vi "Fit To Pane.vi"() -> ()   [LabVIEW 2020]
doc: "Development tool: makes a control fill its pane of a splitter panel and keep filling it (what Fit Control to Pane does by hand). The pane is scrolled to 0,0 and the control moved there; with scaling off, the pane is shrunk to the control's size by moving the two splitter bars that bound it (the window is not resized: writing Panel Bounds answered error 1 once a second pane scaled an object); Scale Single Object is switched on for the control and the bars are put back, so the control grows with the pane and fills it exactly. Works for controls without a writable size (subpanels, multicolumn listboxes). Cell Width > 0 first sizes a multicolumn listbox: the first column's width, one visible column, the number of visible rows, no column headers and no vertical scroll bar; the bars then only make up the last pixels (a bar that would make a pane smaller than its minimum answers error 1358). Height Bar -1: no bar sets the pane's height (a pane beside a vertical bar that runs the full height of the window). Run it on a VI that is not running; it saves the VI (closing the last reference would unload it and drop the changes)."
panel:
  out "error out":errorcluster
  out "pane size":i32[](array[numeric])
  out "control size":i32[](array[numeric])
  in  "Rows":i32
  in  "Row Height":i32
  in  "Cell Width":i32
  in  "Height Bar":i32=1
  in  "Pane Left Of Bar":bool
  in  "Width Bar":i32
  in  "Label":string
  in  "VI":path
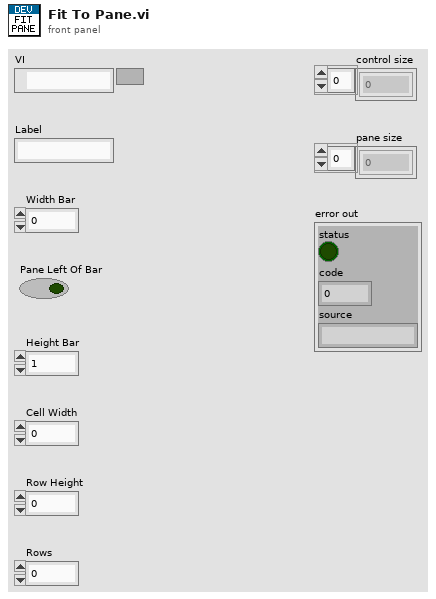
[diagram p1: front panel]
types:
  T1 = enum16{"No Scaling", "Scale All Objects", "Scale Single Object"}
  T2 = typedef "LVBoundsTypeDef.ctl" = cluster{"Width":u32, "Height":u32}
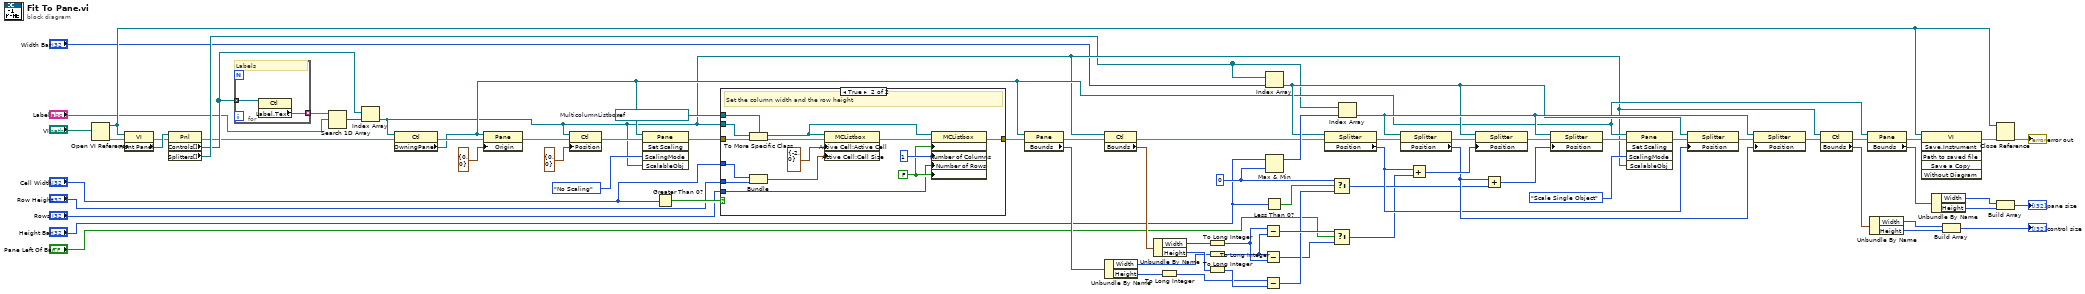
[diagram p0: block diagram]
diagram:
  w63 = refnum<vi> refnum  # MulticolumnListbox
  w46 = 0
  n1 = Open VI Reference(vi path="VI") -> (vi reference=w9:refnum<vi>, error out=w10:errorcluster)  [unwired: 5 in]
  n2 = property class="VI"(reference=w9, error in=w10) -> (error out=w11:errorcluster, "Front Panel"=w12:refnum<vi>)  [unwired: 1 out]
  n3 = property class="Pnl"(reference=w12, error in=w11) -> (error out=w13:errorcluster, "Controls[]"=w14:refnum<vi>[], "Splitters[]"=w15:refnum<vi>[])  [unwired: 1 out]
  n4 = for {
    tunnel: w14 -> [w76] mode=indexing
    tunnel: [w77] -> w16 mode=indexing
    # "Labels"
    n5 = property class="Ctl"(reference=w76) -> ("Label.Text"=w77:string)  [unwired: 1 in, 2 out]
  }
  n6 = Search 1D Array(1D array=w16, element="Label") -> (index of element=w17:i32)  [unwired: 1 in]
  n7 = Index Array(array=w14, index=w17) -> (element=w18:refnum<vi>)
  n8 = property class="Ctl"(reference=w18, error in=w13) -> (error out=w20:errorcluster, "OwningPane"=w19:refnum<vi>)  [unwired: 1 out]
  n9 = property class="Pane"(reference=w19, error in=w20, "Origin"=cluster{"Horizontal":i16, "Vertical":i16} {"Horizontal"=0, "Vertical"=0}) -> (error out=w22:errorcluster)  [unwired: 1 out]
  n10 = property class="Ctl"(reference=w18, error in=w22, "Position"=cluster{"Left":i32, "Top":i32} {"Left"=0, "Top"=0}) -> (error out=w24:errorcluster)  [unwired: 1 out]
  n11 = invoke class="Pane" method="Set Scaling"(reference=w19, error in=w24, "ScalingMode"=T1."No Scaling", "ScalableObj"=w18) -> (error out=w27:errorcluster)  [unwired: 1 in, 4 out]
  n12 = Greater Than 0?(x="Cell Width") -> (x > 0?=w62:bool)
  n13 = case shown="True" w62 {
    tunnel: w63 -> [_ w81]
    tunnel: "Cell Width" -> [_ w82]
    tunnel: "Row Height" -> [_ w83]
    tunnel: "Rows" -> [_ w84]
    tunnel: w18 -> [_ w80]
    tunnel: w27 -> [w78 w79]
    tunnel: [w78 w92] -> w30
    frame False {
      # "Keep them"
    }
    frame True {
      w90 = FALSE
      # "Set the column width and the row height"
      n14 = To More Specific Class(target class=w81, reference=w80, error in=w79) -> (specific class reference=w85:refnum<vi>, error out=w86:errorcluster)
      n15 = Bundle("Cell Width"=w82, "Row Height"=w83) -> (w88:cluster{"Cell Width":i32, "Row Height":i32})  [unwired: 1 in]
      n16 = property class="MCListbox"(reference=w85, error in=w86, "Active Cell:Active Cell"=cluster{"Row":i32, "Column":i32} {"Row"=-2, "Column"=0}, "Active Cell:Cell Size"=w88) -> (error out=w89:errorcluster)  [unwired: 1 out]
      n17 = property class="MCListbox"(reference=w85, error in=w89, "Visible Items:Column Headers Visible"=w90, "Number of Columns"=1, "Number of Rows"=w84, "Visible Items:Vertical Scrollbar Visible"=w90) -> (error out=w92:errorcluster)  [unwired: 1 out]
    }
  }
  n18 = property class="Pane"(reference=w19, error in=w30) -> (error out=w28:errorcluster, "Bounds"=w29:T2)  [unwired: 1 out]
  n19 = Unbundle By Name(w29) -> ("Width"=w33:u32, "Height"=w34:u32)
  n20 = property class="Ctl"(reference=w18, error in=w28) -> (error out=w31:errorcluster, "Bounds"=w32:T2)  [unwired: 1 out]
  n21 = Unbundle By Name(w32) -> ("Width"=w35:u32, "Height"=w36:u32)
  n22 = To Long Integer(number=w34) -> (32bit integer=w38:i32)
  n23 = To Long Integer(number=w35) -> (32bit integer=w39:i32)
  n24 = To Long Integer(number=w33) -> (32bit integer=w37:i32)
  n25 = To Long Integer(number=w36) -> (32bit integer=w40:i32)
  n26 = Subtract(x=w39, y=w37) -> (x-y=w43:i32)
  n27 = Subtract(x=w37, y=w39) -> (x-y=w41:i32)
  n28 = Subtract(x=w38, y=w40) -> (x-y=w42:i32)
  n29 = Less Than 0?(x="Height Bar") -> (x < 0?=w47:bool)
  n30 = Index Array(array=w15, index="Width Bar") -> (element=w45:refnum<vi>)
  n31 = Max & Min(x="Height Bar", y=w46) -> (max(x,y)=w49:i32)  [unwired: 1 out]
  n32 = property class="Splitter"(reference=w45, error in=w31) -> (error out=w51:errorcluster, "Position"=w52:i32)  [unwired: 1 out]
  n33 = Select(t=w46, s=w47, f=w42) -> (s? t:f=w48:i32)
  n34 = Select(t=w43, s="Pane Left Of Bar", f=w41) -> (s? t:f=w44:i32)
  n35 = Index Array(array=w15, index=w49) -> (element=w50:refnum<vi>)
  n36 = property class="Splitter"(reference=w50, error in=w51) -> (error out=w53:errorcluster, "Position"=w54:i32)  [unwired: 1 out]
  n37 = Add(x=w52, y=w44) -> (x+y=w55:i32)
  n38 = property class="Splitter"(reference=w45, error in=w53, "Position"=w55) -> (error out=w57:errorcluster)  [unwired: 1 out]
  n39 = Add(x=w54, y=w48) -> (x+y=w56:i32)
  n40 = property class="Splitter"(reference=w50, error in=w57, "Position"=w56) -> (error out=w58:errorcluster)  [unwired: 1 out]
  n41 = invoke class="Pane" method="Set Scaling"(reference=w19, error in=w58, "ScalingMode"=T1."Scale Single Object", "ScalableObj"=w18) -> (error out=w59:errorcluster)  [unwired: 1 in, 4 out]
  n42 = property class="Splitter"(reference=w45, error in=w59, "Position"=w52) -> (error out=w60:errorcluster)  [unwired: 1 out]
  n43 = property class="Splitter"(reference=w50, error in=w60, "Position"=w54) -> (error out=w61:errorcluster)  [unwired: 1 out]
  n44 = property class="Ctl"(reference=w18, error in=w61) -> (error out=w64:errorcluster, "Bounds"=w65:T2)  [unwired: 1 out]
  n45 = property class="Pane"(reference=w19, error in=w64) -> (error out=w66:errorcluster, "Bounds"=w67:T2)  [unwired: 1 out]
  n46 = Unbundle By Name(w65) -> ("Width"=w68:u32, "Height"=w69:u32)
  n47 = invoke class="VI" method="Save.Instrument"(reference=w9, error in=w66) -> (error out=w74:errorcluster)  [unwired: 4 in, 5 out]
  n48 = Unbundle By Name(w67) -> ("Width"=w70:u32, "Height"=w71:u32)
  n49 = Build Array(w68, w69) -> (→"control size":u32[])
  n50 = Close Reference(reference=w9, error in (no error)=w74) -> (error out=→"error out":errorcluster)
  n51 = Build Array(w70, w71) -> (→"pane size":u32[])
